vi "SC Run Tool.vi"(8 "error in (no error)":errorcluster, 9 "arguments":string[](array[string])) -> (0 "error out":errorcluster, 1 "output":string, 2 "tool lines":string[](array[string]), 3 "result":string, 4 "result detail":string, 5 "exit code":i32)   [LabVIEW 2023]
doc: "Runs systemcore-deploy (next to this VI) with the given arguments through System Exec: systemcore-deploy.cmd on Windows, sh elsewhere. Returns its human-readable output, its SYSTEMCORE-TOOL lines (without the prefix), the RESULT word and detail, and its exit code."
uses:
  <vilib>/Utility/error.llb/Trim Whitespace One-Sided.vi
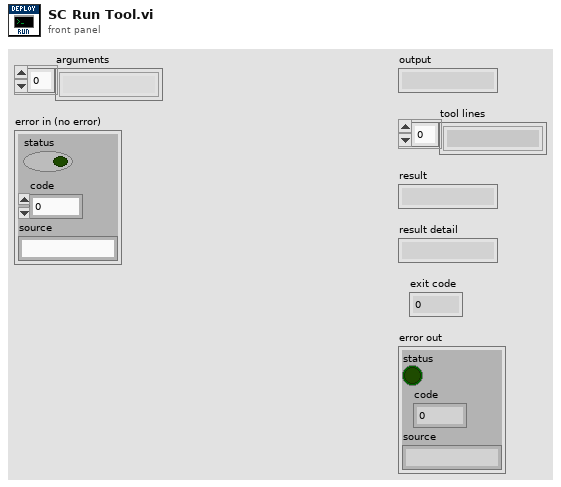
[diagram p1: front panel]
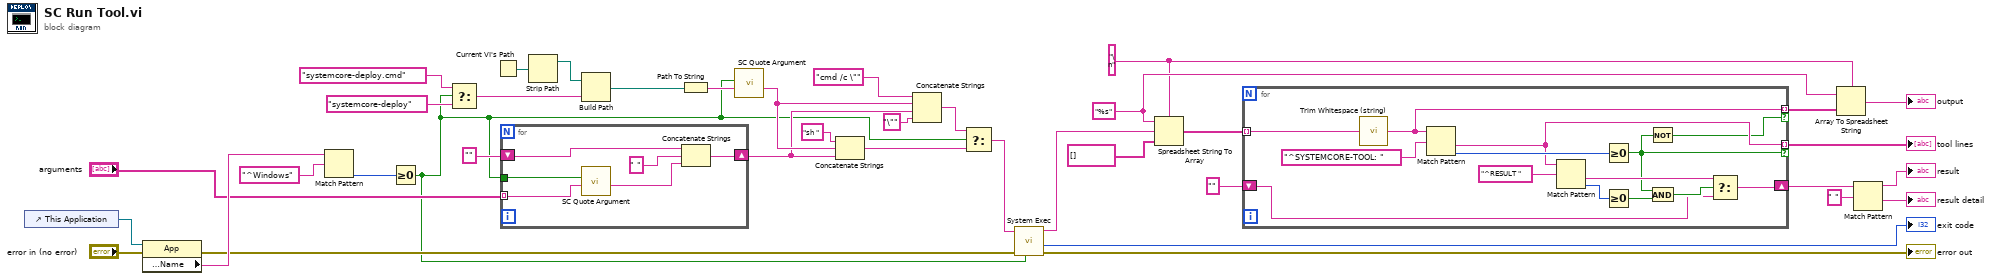
[diagram p0: block diagram]
diagram:
  w6 = "\n"
  w8 = "%s"
  n1 = control-ref of="This Application"() -> (w39:refnum<vi>)
  n2 = property class="App"(reference=w39, error in="error in (no error)") -> (error out=w17:errorcluster, "Operating System:Name"=w37:string)  [unwired: 1 out]
  n3 = Match Pattern(string=w37, regular expression="^Windows") -> (offset past match=w35:i32)  [unwired: 1 in, 3 out]
  n4 = Greater Or Equal To 0?(x=w35) -> (x >= 0?=w16:bool)
  n5 = Select(t="systemcore-deploy.cmd", s=w16, f="systemcore-deploy") -> (s? t:f=w30:string)
  n6 = Current VI's Path() -> (path=w34:path)
  n7 = for {
    tunnel: "arguments" -> [w45] mode=indexing
    tunnel: w16 -> [w44]
    shift-right: [w40] -> w21
    shift-left: "" -> [w43]
    n8 = call "SC Quote Argument.vi"("argument"=w45, "windows?"=w44) -> ("quoted argument"=w41:string)  [unwired: 9 in]
    n9 = Concatenate Strings(w43, " ", w41) -> (w40:string)
  }
  n10 = Strip Path(path=w34) -> (stripped path=w31:path)  [unwired: 1 out]
  n11 = Build Path(base path=w31, name or relative path=w30) -> (appended path=w29:path)
  n12 = Path To String(path=w29) -> (string=w28:string)
  n13 = call "SC Quote Argument.vi"("argument"=w28, "windows?"=w16) -> ("quoted argument"=w22:string)  [unwired: 9 in]
  n14 = Concatenate Strings("sh ", w22, w21) -> (w19:string)
  n15 = Concatenate Strings("cmd /c \"", w22, w21, "\"") -> (w20:string)
  n16 = Select(t=w20, s=w16, f=w19) -> (s? t:f=w18:string)
  n17 = call <vilib>:"System Exec.vi"("run minimized? (F)"=w16, "error in (no error)"=w17, "command line"=w18) -> ("error out"=→"error out":errorcluster, "return code"=→"exit code":i32, "standard output"=w13:string)  [unwired: 5 in, 1 out]
  n18 = Spreadsheet String To Array(delimiter (Tab)=w6, format string=w8, spreadsheet string=w13, array type (2D Dbl)=string[] []) -> (array=w11:string[])
  n19 = for {
    tunnel: w11 -> [w59] mode=indexing
    shift-right: [w50] -> w4
    shift-left: "" -> [w51]
    tunnel: [w48] -> w9 mode=indexing if=w49
    tunnel: [w46] -> w7 mode=indexing if=w47
    n20 = call <vilib>:"Trim Whitespace (string).vi"("string"=w59) -> ("trimmed string"=w46:string)  [unwired: 1 in]
    n21 = Match Pattern(string=w46, regular expression="^SYSTEMCORE-TOOL: ") -> (after substring=w48:string, offset past match=w57:i32)  [unwired: 1 in, 2 out]
    n22 = Match Pattern(string=w48, regular expression="^RESULT ") -> (after substring=w52:string, offset past match=w55:i32)  [unwired: 1 in, 2 out]
    n23 = Greater Or Equal To 0?(x=w57) -> (x >= 0?=w49:bool)
    n24 = Greater Or Equal To 0?(x=w55) -> (x >= 0?=w54:bool)
    n25 = Not(x=w49) -> (.not. x?=w47:bool)
    n26 = And(x=w49, y=w54) -> (x .and. y?=w53:bool)
    n27 = Select(t=w52, s=w53, f=w51) -> (s? t:f=w50:string)
  }
  "tool lines" <- w9
  n28 = Array To Spreadsheet String(delimiter (Tab)=w6, array=w7, 3:w8) -> (spreadsheet string=→"output":string)
  n29 = Match Pattern(string=w4, regular expression=" ") -> (before substring=→"result":string, after substring=→"result detail":string)  [unwired: 1 in, 2 out]
